vi "Dmtch Add Strategy.vi"(0 "nIndex":i32, 1 "times":sgl, 2 "fFreq":sgl, 5 "nStr":i32[](array[numeric])=array[4097 elements], 7 "nNum":i32, 9 "nWinLen":u64, 11 "error in (no error)":errorcluster caption="错误输入（无错误）", 12 "nRes":i32, 13 "nDataType":i32) -> (4 "function return":i32, 6 "nStr out":i32[](array[numeric]), 15 "error out":errorcluster caption="错误输出")   [LabVIEW 2017, in "smncsftmt.lvlib"]
doc: "__declspec(dllexport) int DmtchAddStrategy(int nIndex, int nStr[], int nNum, unsigned long long nWinLen, float times, int nRes = 0, float fFreq = 0.0f, int nDataType = 0);"
uses:
  smncsftmt.lvlib
  smncsftmt.dll
panel:
  # "s"
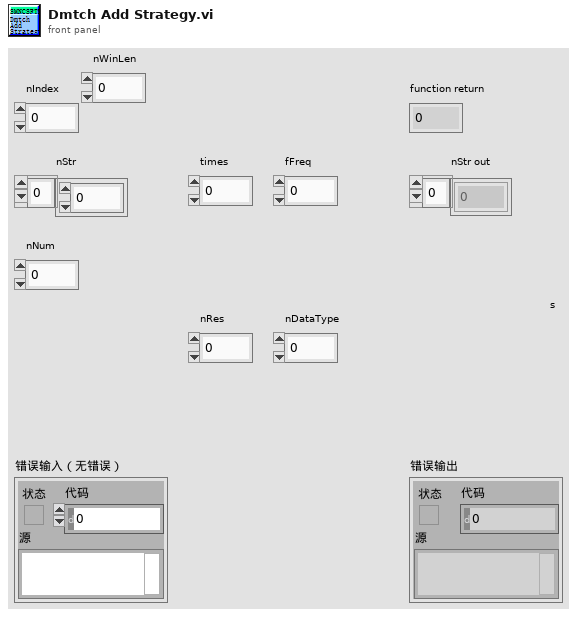
[diagram p1: front panel]
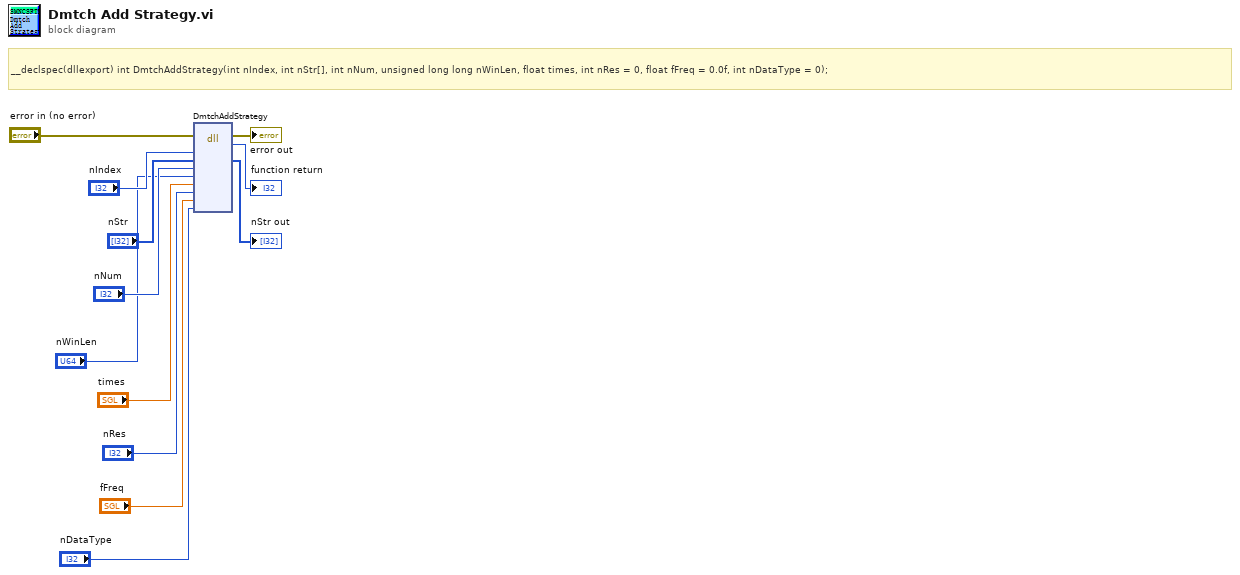
[diagram p0: block diagram]
diagram:
  # "__declspec(dllexport) int DmtchAddStrategy(int nIndex, int nStr[], int nNum, unsigned long long nWinLen, float times, int nRes = 0, float fFreq = 0.0f, int nDataType = 0);"
  n1 = dll-call lib="PTH2oabs CUsersaDesktop\nLABVIEW范例National InstrumentsLabVIEW 2017user.lib\tsmncsftmtsmncsftmt.*" fn="DmtchAddStrategy"(error in="error in (no error)", "nIndex"="nIndex", "nStr"="nStr", "nNum"="nNum", "nWinLen"="nWinLen", "times"="times", "nRes"="nRes", "fFreq"="fFreq", "nDataType"="nDataType") -> (error out=→"error out":errorcluster, "返回类型"=→"function return":i32, "nStr"=→"nStr out":i32[])  [unwired: 9 in, 1 out]
